vi "GetConfigurationType.vi"(8 "error in (no error)":errorcluster, 11 "object in":refnum<class "AIO_Channel.lvclass">) -> (0 "error out":errorcluster, 2 "Configuration":refnum<class "Configuration.lvclass">, 3 "object out":refnum<class "AIO_Channel.lvclass">)   [LabVIEW 2021, in "DAQmx.lvlib" / "AIO_Channel.lvclass"]
doc: "Gets the Configuration to use"
uses:
  AIO_Channel.lvclass
  Dependencies/Channel.lvlibp/Channel/Configuration_class/Configuration.lvclass
  AIO-Configuration_class/AIO-Configuration.lvclass
  C:/Users/averna/Documents/LV Gym DEMO/Factory Pattern/Device Channels/Dependencies/Channel.lvlibp/Channel/Configuration_class/Configuration.lvclass
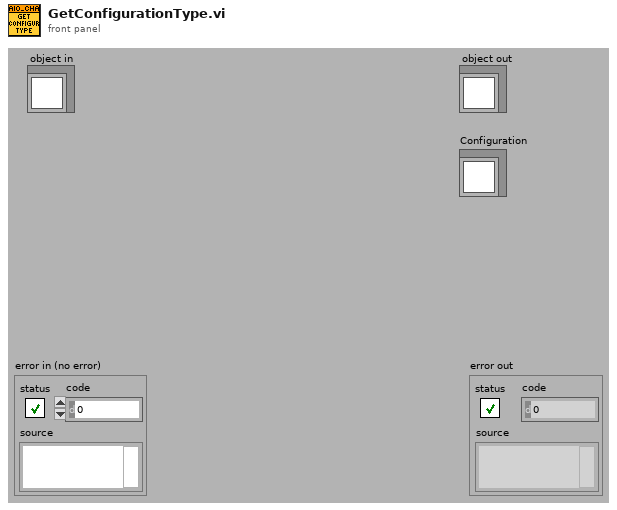
[diagram p1: front panel]
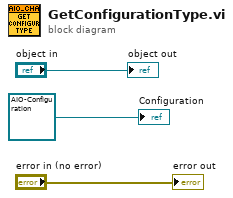
[diagram p0: block diagram]
diagram:
  "error out" <- "error in (no error)"
  "object out" <- "object in"
  "Configuration" <- refnum<class "AIO-Configuration.lvclass"> refnum ("DAQmx.lvlib:AIO_CFG")
